vi "Validate Sequence.vi"(8 "error in":errorcluster, 10 "Rig Config":T1, 11 "Sequence File":T3) -> (0 "error out":errorcluster, 2 "problems":string[](array[string]), 3 "valid":bool=TRUE)   [LabVIEW 2026]
doc: "Validates a Sequence File against a Rig Config: every setpoint and condition channel must exist in the rig, every setpoint value must be within the channel min/max, every condition tolerance must be >= 0, and every timeout_ms must be > 0. Returns a problems string array (empty means valid) and a valid flag; it does NOT return an error for invalid sequences. AF-free."
uses:
  Typedefs/Condition.ctl
  Typedefs/Channel Value.ctl
  Typedefs/Step Config.ctl
  Typedefs/Sequence File.ctl
  Typedefs/Channel Definition.ctl
  Typedefs/Rig Config.ctl
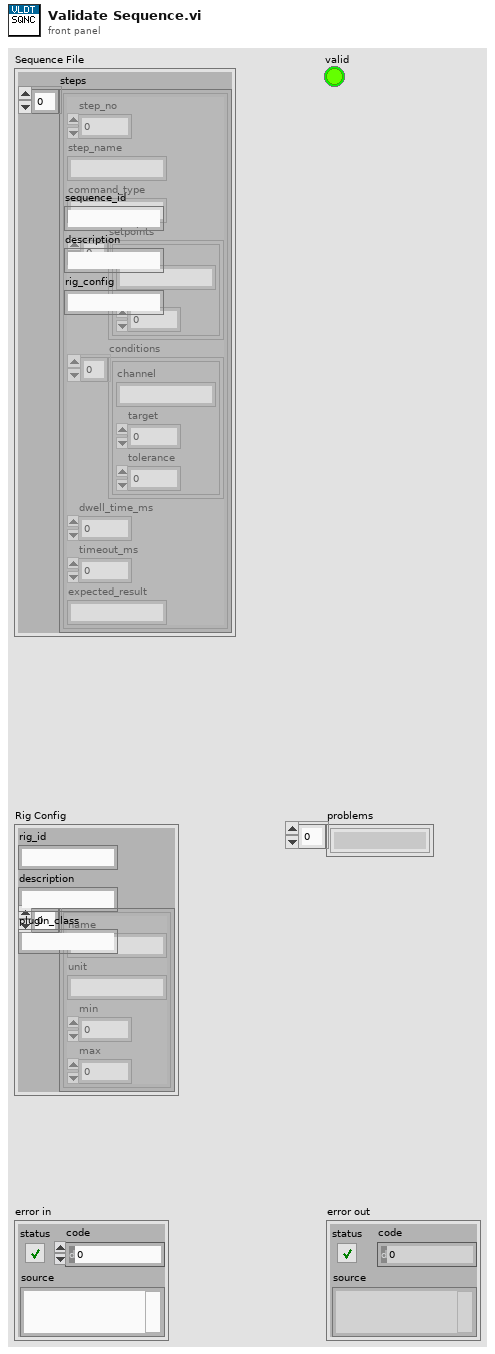
[diagram p1: front panel]
types:
  T1 = typedef "Rig Config.ctl" = cluster{"rig_id":string, "description":string, "plugin_class":string, "channels":T2[]}
  T2 = typedef "Channel Definition.ctl" = cluster{"name":string, "unit":string, "min":dbl, "max":dbl}
  T3 = typedef "Sequence File.ctl" = cluster{"sequence_id":string, "description":string, "rig_config":string, "steps":T4[]}
  T4 = typedef "Step Config.ctl" = cluster{"step_no":i32, "step_name":string, "command_type":string, "setpoints":T5[], "conditions":T6[], "dwell_time_ms":i32, "timeout_ms":i32, "expected_result":string}
  T5 = typedef "Channel Value.ctl" = cluster{"channel":string, "value":dbl}
  T6 = typedef "Condition.ctl" = cluster{"channel":string, "target":dbl, "tolerance":dbl}
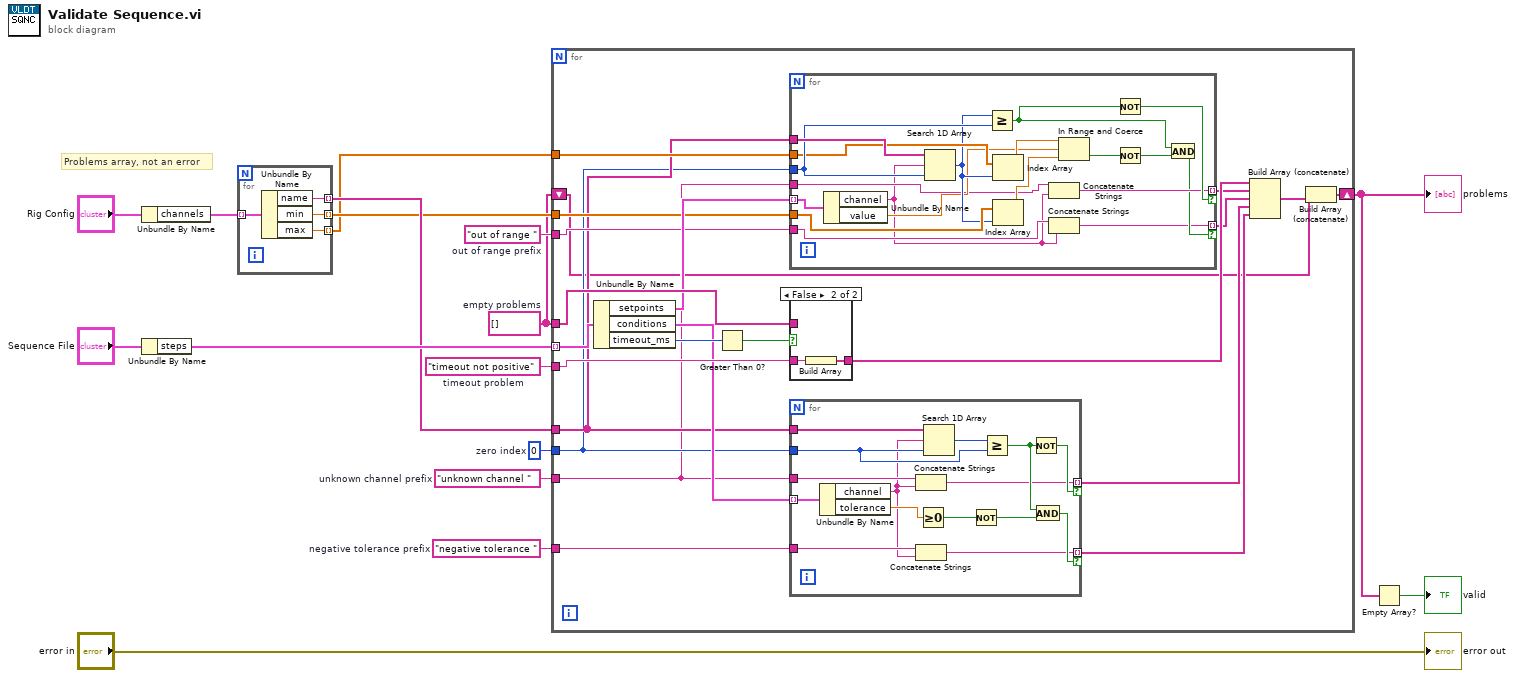
[diagram p0: block diagram]
diagram:
  w5 = "timeout not positive"  # timeout problem
  w6 = "negative tolerance "  # negative tolerance prefix
  w7 = "out of range "  # out of range prefix
  w8 = "unknown channel "  # unknown channel prefix
  w4 = string[] []  # empty problems
  w9 = 0  # zero index
  # "Problems array, not an error"
  n1 = Unbundle By Name("Rig Config") -> ("channels"=w14:T2[])
  n2 = Unbundle By Name("Sequence File") -> ("steps"=w13:T4[])
  n3 = for {
    tunnel: w14 -> [w20] mode=indexing
    tunnel: [w19] -> w12 mode=indexing
    tunnel: [w18] -> w11 mode=indexing
    tunnel: [w17] -> w10 mode=indexing
    n4 = Unbundle By Name(w20) -> ("name"=w19:string, "min"=w18:dbl, "max"=w17:dbl)
  }
  n5 = for {
    tunnel: w13 -> [w42] mode=indexing
    tunnel: w12 -> [w32]
    tunnel: w11 -> [w36]
    tunnel: w10 -> [w35]
    tunnel: w9 -> [w31]
    tunnel: w4 -> [w40]
    tunnel: w8 -> [w30]
    tunnel: w7 -> [w34]
    tunnel: w6 -> [w29]
    tunnel: w5 -> [w39]
    shift-right: [w21] -> w2
    shift-left: w4 -> [w23]
    n6 = Unbundle By Name(w42) -> ("setpoints"=w37:T5[], "conditions"=w33:T6[], "timeout_ms"=w41:i32)
    n7 = Greater Than 0?(x=w41) -> (x > 0?=w38:bool)
    n8 = for {
      tunnel: w37 -> [w76] mode=indexing
      tunnel: w32 -> [w75]
      tunnel: w36 -> [w73]
      tunnel: w35 -> [w72]
      tunnel: w31 -> [w74]
      tunnel: w30 -> [w64]
      tunnel: w34 -> [w63]
      tunnel: [w60] -> w27 mode=indexing if=w61
      tunnel: [w58] -> w26 mode=indexing if=w59
      n9 = Unbundle By Name(w76) -> ("channel"=w62:string, "value"=w69:dbl)
      n10 = Search 1D Array(1D array=w75, element=w62, start index (0)=w74) -> (index of element=w71:i32)
      n11 = Greater Or Equal?(x=w71, y=w74) -> (x >= y?=w66:bool)
      n12 = Index Array(array=w72, index=w71) -> (element=w70:dbl)
      n13 = Index Array(array=w73, index=w71) -> (element=w68:dbl)
      n14 = Concatenate Strings(w64, w62) -> (w60:string)
      n15 = Concatenate Strings(w63, w62) -> (w58:string)
      n16 = In Range and Coerce(upper limit=w70, x=w69, lower limit=w68) -> (In Range?=w67:bool)  [unwired: 1 out]
      n17 = Not(x=w66) -> (.not. x?=w61:bool)
      n18 = Not(x=w67) -> (.not. x?=w65:bool)
      n19 = And(x=w66, y=w65) -> (x .and. y?=w59:bool)
    }
    n20 = case shown="False" w38 {
      tunnel: [w77 w78] -> w28
      tunnel: w40 -> [w77 _]
      tunnel: w39 -> [_ w79]
      frame True {
      }
      frame False {
        n21 = Build Array(w79) -> (w78:string[])
      }
    }
    n22 = for {
      tunnel: w33 -> [w57] mode=indexing
      tunnel: w32 -> [w56]
      tunnel: w31 -> [w54]
      tunnel: w30 -> [w49]
      tunnel: w29 -> [w48]
      tunnel: [w45] -> w25 mode=indexing if=w46
      tunnel: [w43] -> w24 mode=indexing if=w44
      n23 = Unbundle By Name(w57) -> ("channel"=w47:string, "tolerance"=w53:dbl)
      n24 = Concatenate Strings(w49, w47) -> (w45:string)
      n25 = Concatenate Strings(w48, w47) -> (w43:string)
      n26 = Greater Or Equal To 0?(x=w53) -> (x >= 0?=w52:bool)
      n27 = Search 1D Array(1D array=w56, element=w47, start index (0)=w54) -> (index of element=w55:i32)
      n28 = Not(x=w52) -> (.not. x?=w50:bool)
      n29 = Greater Or Equal?(x=w55, y=w54) -> (x >= y?=w51:bool)
      n30 = Not(x=w51) -> (.not. x?=w46:bool)
      n31 = And(x=w51, y=w50) -> (x .and. y?=w44:bool)
    }
    n32 = Build Array (concatenate)(w28, w27, w26, w25, w24) -> (w22:string[])
    n33 = Build Array (concatenate)(w23, w22) -> (w21:string[])
  }
  "problems" <- w2
  n34 = Empty Array?(array=w2) -> (empty?=→"valid":bool)
  "error out" <- "error in"
